vi "lvmcp_server.vi"() -> ()   [LabVIEW 2014]
panel:
  in  "port":u16=5577
  in  "listen address":string="127.0.0.1"
  in  "token":string
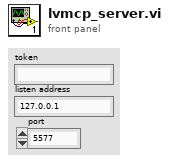
[diagram p1: front panel]
types:
  T1 = enum16{"Standard", "Buffered", "CRLF", "Immediate"}
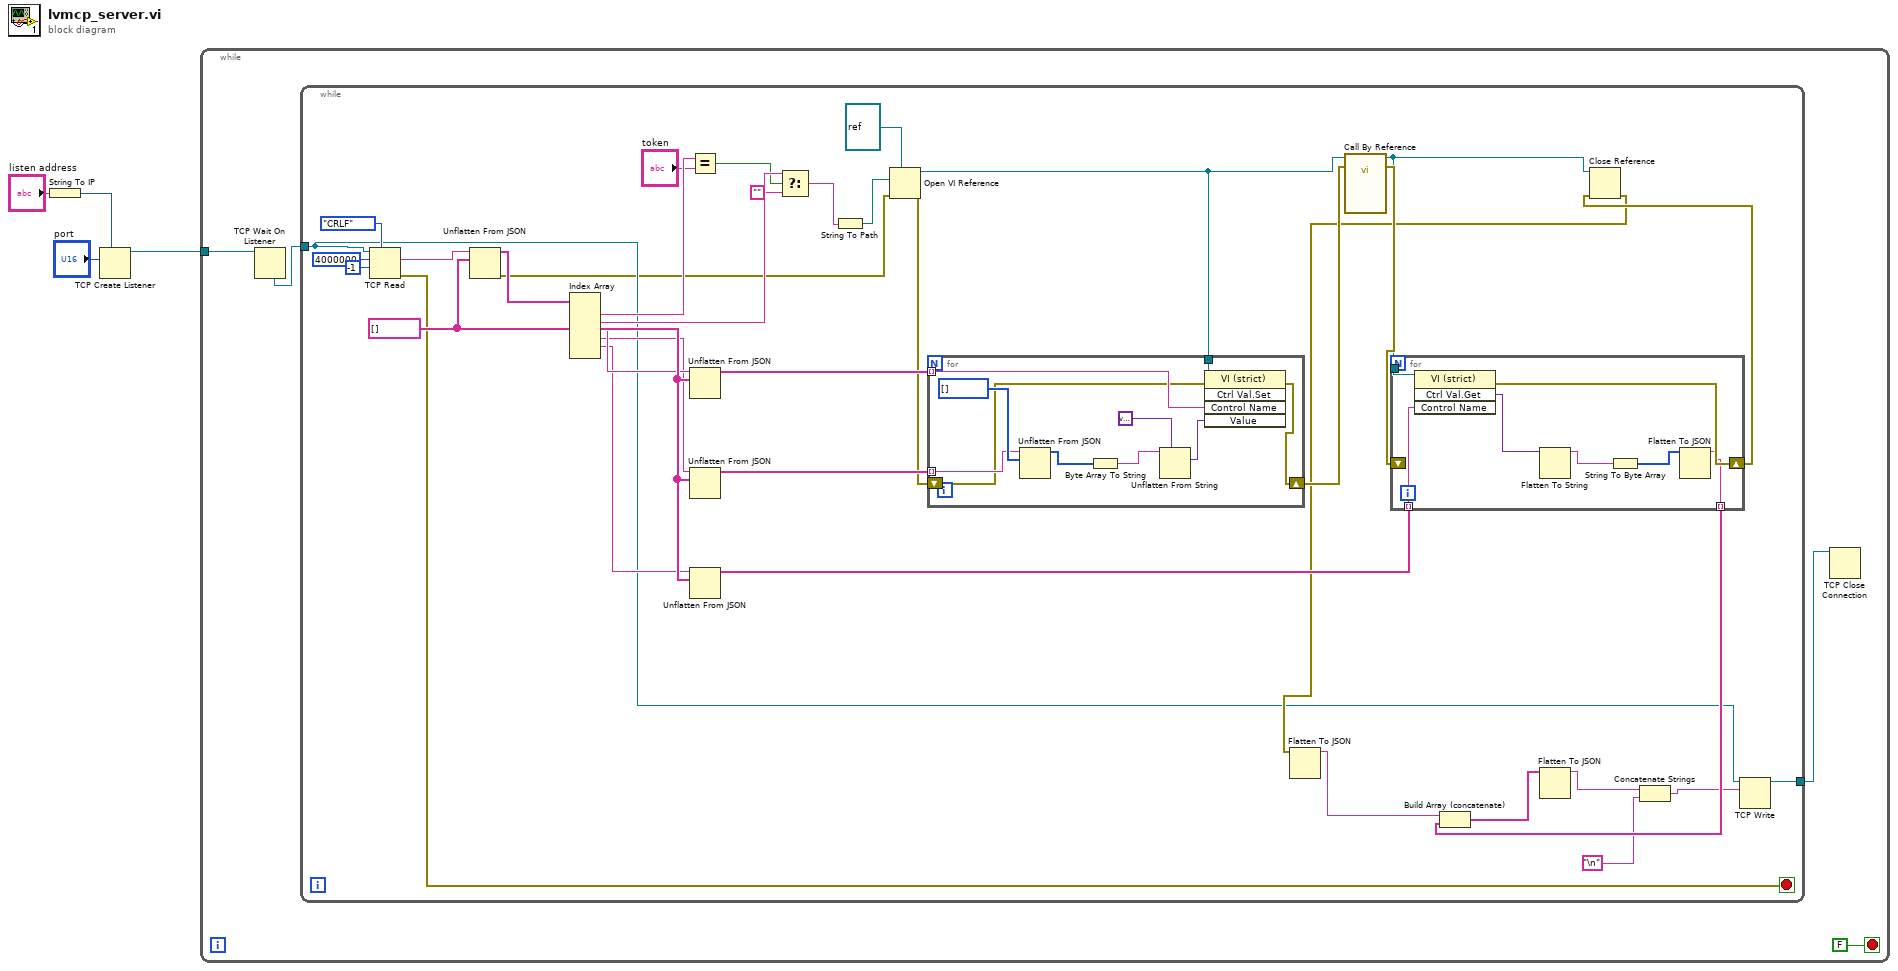
[diagram p0: block diagram]
diagram:
  n1 = String To IP(1:"listen address") -> (0:w3:u32)
  n2 = TCP Create Listener(7:w3, 10:"port") -> (3:w4:refnum<k5>)  [unwired: 3 in, 2 out]
  n3 = while {
    tunnel: w4 -> [w8]
    stop <- FALSE stop-if-true
    n4 = TCP Wait On Listener(11:w8) -> (4:w7:refnum<k5>)  [unwired: 3 in, 4 out]
    n5 = while {
      tunnel: w7 -> [w14]
      tunnel: [w12] -> w5
      stop <- w13 stop-if-true
      w43 = string[] []
      n6 = TCP Read(connection ID=w14, bytes to read=4000000, 7:T1."CRLF" ("mode (standard)"), 9:-1 ("timeout ms (25000)")) -> (data out=w45:string, error out=w13:errorcluster)  [unwired: 1 in, 1 out]
      n7 = Unflatten From JSON(JSON string=w45, type and defaults=w43) -> (value=w44:string[], error out=w11:errorcluster)  [unwired: 5 in]
      n8 = Index Array(array=w44) -> (element #1=w42:string, element #2=w41:string, element #3=w39:string, element #4=w38:string, element #5=w37:string)  [unwired: 6 in, 1 out]
      n9 = Equal?(x=w42, y="token") -> (x = y?=w40:bool)
      n10 = Unflatten From JSON(JSON string=w39, type and defaults=w43) -> (value=w32:string[])  [unwired: 5 in, 1 out]
      n11 = Unflatten From JSON(JSON string=w38, type and defaults=w43) -> (value=w31:string[])  [unwired: 5 in, 1 out]
      n12 = Unflatten From JSON(JSON string=w37, type and defaults=w43) -> (value=w28:string[])  [unwired: 5 in, 1 out]
      n13 = Select(t=w41, s=w40, f="") -> (s? t:f=w10:string)
      n14 = String To Path(string=w10) -> (path=w9:path)
      n15 = Open VI Reference(type specifier VI Refnum (for type only)=refnum<vi> refnum, vi path=w9, error in (no error)=w11) -> (vi reference=w33:refnum<vi>, error out=w30:errorcluster)  [unwired: 3 in]
      n16 = for {
        tunnel: w33 -> [w62]
        tunnel: w32 -> [w59] mode=indexing
        tunnel: w31 -> [w58] mode=indexing
        shift-right: [w53] -> w29
        shift-left: w30 -> [w54]
        n17 = Unflatten From JSON(JSON string=w58, type and defaults=i32[] []) -> (value=w57:i32[])  [unwired: 5 in, 1 out]
        n18 = Byte Array To String(unsigned byte array=w57) -> (string=w56:string)
        n19 = Unflatten From String(type=variant, binary string=w56) -> (value=w55:variant)  [unwired: 3 in, 2 out]
        n20 = invoke class="VI (strict)" method="Ctrl Val.Set"(reference=w62, error in=w54, "Control Name"=w59, "Value"=w55) -> (error out=w53:errorcluster)  [unwired: 1 in, 4 out]
      }
      n21 = call-by-ref "?"(reference=w33, error in=w29) -> (reference out=w25:refnum<vi>, error out=w27:errorcluster)  [unwired: 12 in]
      n22 = for {
        tunnel: w25 -> [w52]
        tunnel: w28 -> [w51] mode=indexing
        shift-right: [w47] -> w26
        shift-left: w27 -> [_]
        tunnel: [w46] -> w22 mode=indexing
        n23 = invoke class="VI (strict)" method="Ctrl Val.Get"(reference=w52, "Control Name"=w51) -> (error out=w47:errorcluster, "Get Control Value Variant"=w50:variant)  [unwired: 2 in, 2 out]
        n24 = Flatten To String(anything=w50) -> (data string=w49:string)  [unwired: 3 in, 2 out]
        n25 = String To Byte Array(string=w49) -> (unsigned byte array=w48:u8[])
        n26 = Flatten To JSON(anything=w48) -> (JSON string=w46:string)  [unwired: 2 in, 1 out]
      }
      n27 = Close Reference(reference=w25, error in (no error)=w26) -> (error out=w24:errorcluster)
      n28 = Flatten To JSON(anything=w24) -> (JSON string=w23:string)  [unwired: 2 in, 1 out]
      n29 = Build Array (concatenate)(w23, w22) -> (w21:string[])
      n30 = Flatten To JSON(anything=w21) -> (JSON string=w20:string)  [unwired: 2 in, 1 out]
      n31 = Concatenate Strings(w20, "\n") -> (w18:string)
      n32 = TCP Write(connection ID=w14, data in=w18) -> (connection ID out=w12:refnum<k5>)  [unwired: 2 in, 2 out]
    }
    n33 = TCP Close Connection(connection ID=w5) -> ()  [unwired: 2 in, 2 out]
  }
